vi "Create AI Resource.vi"(8 "error in (no error)":errorcluster) -> (0 "error out":errorcluster, 2 "found?":bool, 3 "task out":i32)   [LabVIEW 2021]
uses:
  <userlib>/DAQNavi Polymorphic VI/create/DAQNavi Create Channel(AI-Voltage).vi
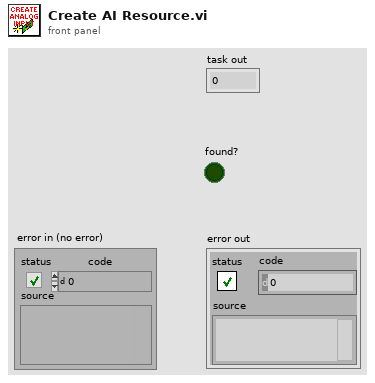
[diagram p1: front panel]
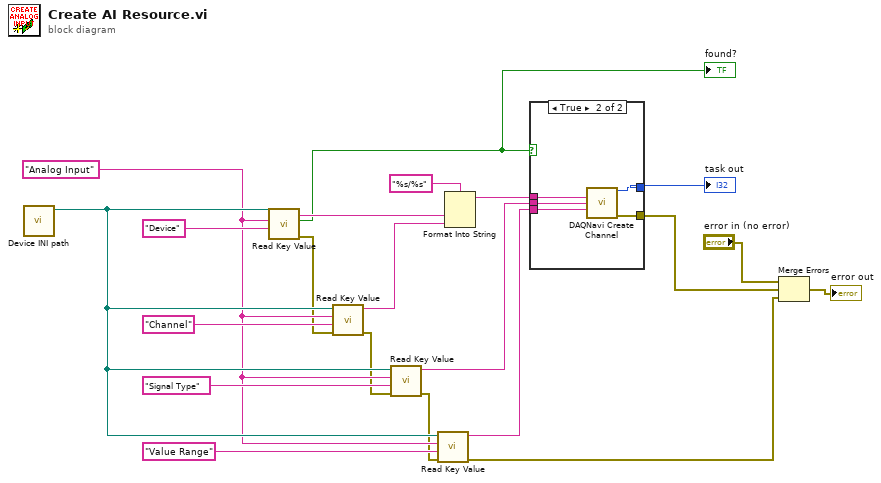
[diagram p0: block diagram]
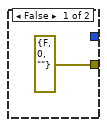
[diagram p2: hidden frame]
diagram:
  w13 = "Analog Input" ("Device Session Name")
  n1 = call "Device INI path.vi"() -> ("appended path"=w14:path)  [unwired: 11 in]
  n2 = call "Read Key Value.vi"("key"="Device", "Device Session Name"=w13, "appended path"=w14) -> ("error out"=w5:errorcluster, "found?"=w8:bool, "value"=w12:string)  [unwired: 6 in]
  "found?" <- w8
  n3 = call "Read Key Value.vi"("error in (no error)"=w5, "key"="Channel", "Device Session Name"=w13, "appended path"=w14) -> ("error out"=w4:errorcluster, "value"=w11:string)  [unwired: 5 in, 1 out]
  n4 = call "Read Key Value.vi"("error in (no error)"=w4, "key"="Signal Type", "Device Session Name"=w13, "appended path"=w14) -> ("error out"=w3:errorcluster, "value"=w10:string)  [unwired: 5 in, 1 out]
  n5 = call "Read Key Value.vi"("error in (no error)"=w3, "key"="Value Range", "Device Session Name"=w13, "appended path"=w14) -> ("error out"=w2:errorcluster, "value"=w9:string)  [unwired: 5 in, 1 out]
  n6 = Format Into String(format string="%s/%s", w12, w11) -> (resulting string=w20:string)  [unwired: 2 in, 1 out]
  n7 = case shown="True" w8 {
    tunnel: w20 -> [_ w27]
    tunnel: [errorcluster {"status"=FALSE, "code"=0, "source"=""} ("error out") w26] -> w6
    tunnel: [_ w25] -> w19
    tunnel: w10 -> [_ w24]
    tunnel: w9 -> [_ w23]
    frame False {
    }
    frame True {
      n8 = call-poly <userlib>:"DAQNavi Create Channel.vi"("physical channels"=w27, "signal type"=w24, "value range"=w23) -> ("task out"=w25:i32, "error out"=w26:errorcluster)  [unwired: 11 in]
    }
  }
  "task out" <- w19
  n9 = Merge Errors("error in (no error)", w6, w2) -> (→"error out":errorcluster)
